vi "Dashboard Main.vi"() -> ()   [LabVIEW 2013]
uses:
  <vilib>/event_ctls.llb/eventvkey.ctl
  <vilib>/Rock Robotics/WPI/Dashboard/WPI_DashboardLogging Global.vi
  <vilib>/Utility/config.llb/Write Key (String).vi
  <vilib>/Utility/config.llb/Write Key (I32).vi
  <vilib>/Utility/config.llb/NI_LVConfig.lvlib
panel:
  out "Image Message":string="Timeout in Camera Communications"
  in  "Rec Mode":enum32{"Stop", "Record", "Playback"}(radio)
  in  "Dashboard Tab":T1(tab)
  out "Error":bool
  in  "Camera Settings":T2={"Frame Rate"=30, "Compression"=30, "Size"=1} {"Frame Rate" scale=1.0..30.0; "Size" items=["640x480", "320x240", "160x120"]}
  out "MotorSliders R":cluster{"MotorSlide1":dbl, "MotorSlide2":dbl} {"MotorSlide2" scale=-1.0..1.0 scale format="%#_2e"; "MotorSlide1" scale=-1.0..1.0 scale format="%#_2e"}
  out "MotorChart R":cluster{"Numeric":dbl, "Numeric":dbl}(graph)
  out "MotorSliders L":T3 {"MotorSlide4 2" scale=0.0..14.0 scale format="%#_2e"; "MotorSlide2" scale=-1.0..1.0 scale format="%#_2e"; "MotorSlide1" scale=-1.0..1.0 scale format="%#_2e"}
  out "MotorChart L":T4(graph)
  out "JS1 Z":dbl(slide) scale=-1.0..1.0 scale format="%#_2e"
  out "Joystick 1":cluster{"X":dbl, "Y":dbl}[](graph)
  out "JS Buttons 1":T5
  out "JS2 Z":dbl(slide) scale=-1.0..1.0 scale format="%#_2e"
  out "Joystick 2":cluster{"X":dbl, "Y":dbl}[](graph)
  out "JS Buttons 2":T5
  out "Mode":T6(ring)=enum."Auto Disabled"
  out "Camera IP":string
  in  "DB Camera Config":bool
  out "fps":dbl format="%#.1g"
  out "Mbps":dbl format="%#.1g"
  out "Mbps 2":bool
  in  "Test Slider":dbl(slide) scale=0.0..100.0 scale format="%#_3g"
  in  "On/Off":bool caption="Solenoid"
  in  "Test Name":u16(ring) items=["Select the test to run...", "Example Test", "-------------------------------", "List of tests is built in robot code.", "Replace with your own automated tests."]
  in  "Test Tree":string(tree)
  in  "Motor":cluster{"Value":dbl, "Enable":bool} {"Value" scale=-1.0..1.0 scale format="%#_3g"}
  out "Progress":T7 {"Test Progress" scale=0.0..100.0}
  in  "Rev/Fwd":cluster{"Forward":bool, "Reverse":bool}
  in  "Test Ring":u16(ring) items=["Auto", "Fixed indoor", "Fixed outdoor 1", "Fixed outdoor 2", "Fixed fluorescent 1", "Fixed fluorescent 2", "Hold current"]
  in  "Listbox":i32(listbox)
  out "Tree":string(tree)
  in  "Reset":bool
  out "Errors":T8(array[cluster])
  out "Camera Image":T9(plugin-control)
  in  "Enable":bool
  # "Left"
  # "Front"
  # "Right"
  # "Battery"
  # "Customize by placing controls and indicators here and name to\nmatch Dashboard Variables on robot."
  # "This tab is a great place for autonomous settings and validation.\nCustomize by placing controls and indicators here and name to\nmatch Dashboard Variables on robot."
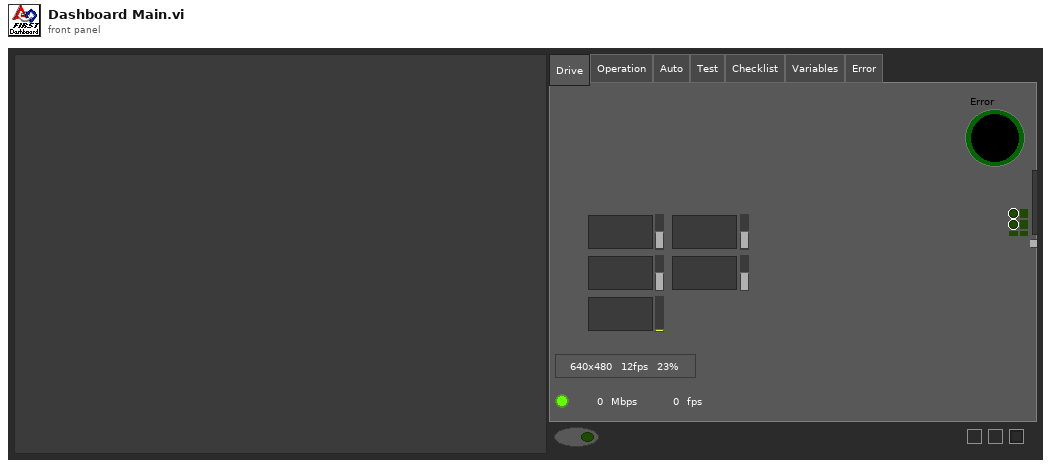
[diagram p1: front panel]
types:
  T1 = enum32{"Drive", "Operation", "Auto", "Test", "Checklist", "Variables", "Error"}
  T2 = cluster{"Frame Rate":i32, "Compression":i32, "Size":u16}
  T3 = cluster{"MotorSlide1":dbl, "MotorSlide2":dbl, "MotorSlide4 2":dbl}
  T4 = cluster{"Numeric":dbl, "Numeric":dbl, "Battery":sgl}
  T5 = cluster{bool, bool, bool, bool, bool, bool, bool, bool, bool, bool, bool, bool}
  T6 = enum8{"Tele-Op Disabled", "Tele-Op Enabled", "Auto Disabled", "Auto Enabled", "Test Disabled", "Test Enabled", ""}
  T7 = cluster{"Test Progress":u8, "Test Progress Text":string}
  T8 = cluster{"status":bool, "code":i32, "location":string, "source":string}[]
  T9 = typedef "IMAQ Image.ctl" = refnum<image>
  T10 = enum32{"Drive", "Operation", "Auto", "Test", "Checklist", "Variables"}
  T11 = typedef "Image Type" = u32
  T12 = cluster{"Digital Inputs":bool[], "Digital Outputs":bool[]}
  T13 = cluster{"Competition mode":bool, "Robot Link":bool, "Autonomous":bool, "Enabled":bool, "E-Stop":bool, "Simulated":bool, "TestMode":bool, "Docked Window":bool}
  T14 = cluster{"Boolean":bool, "Numeric":i32, "String":string, "String":string}[]
  T15 = typedef "NI_LVConfig.lvlib/Config Data RefNum.ctl" = refnum<k1>
  T16 = typedef "eventvkey.ctl" = enum16{"ASCII", "Enter", "Return", "Shift", "Ctrl", "Alt", "Cmd", "Opt", "Caps", "NumLock", "Clear", "Break", "Up", "Down", "Left", "Right", "Insert", "Delete", "Home", "End", "PageUp", "PageDown", "Escape", "Help", "Pause", "ScrollLock", "F1", "F2", "F3", "F4", "F5", "F6", "F7", "F8", "F9", "F10", "F11", "F12", "F13", "F14", "F15", "F16", "F17", "F18", "F19", "F20", "F21", "F22", "F23", "F24", "Play", "VolumeUp", "VolumeDown", "Mute", "Two Byte Char"}
  T17 = cluster{"Image Size":bool, "Image Type":bool, "Pixel Value":bool, "ROI Information":bool, "Zoom Factor":bool}
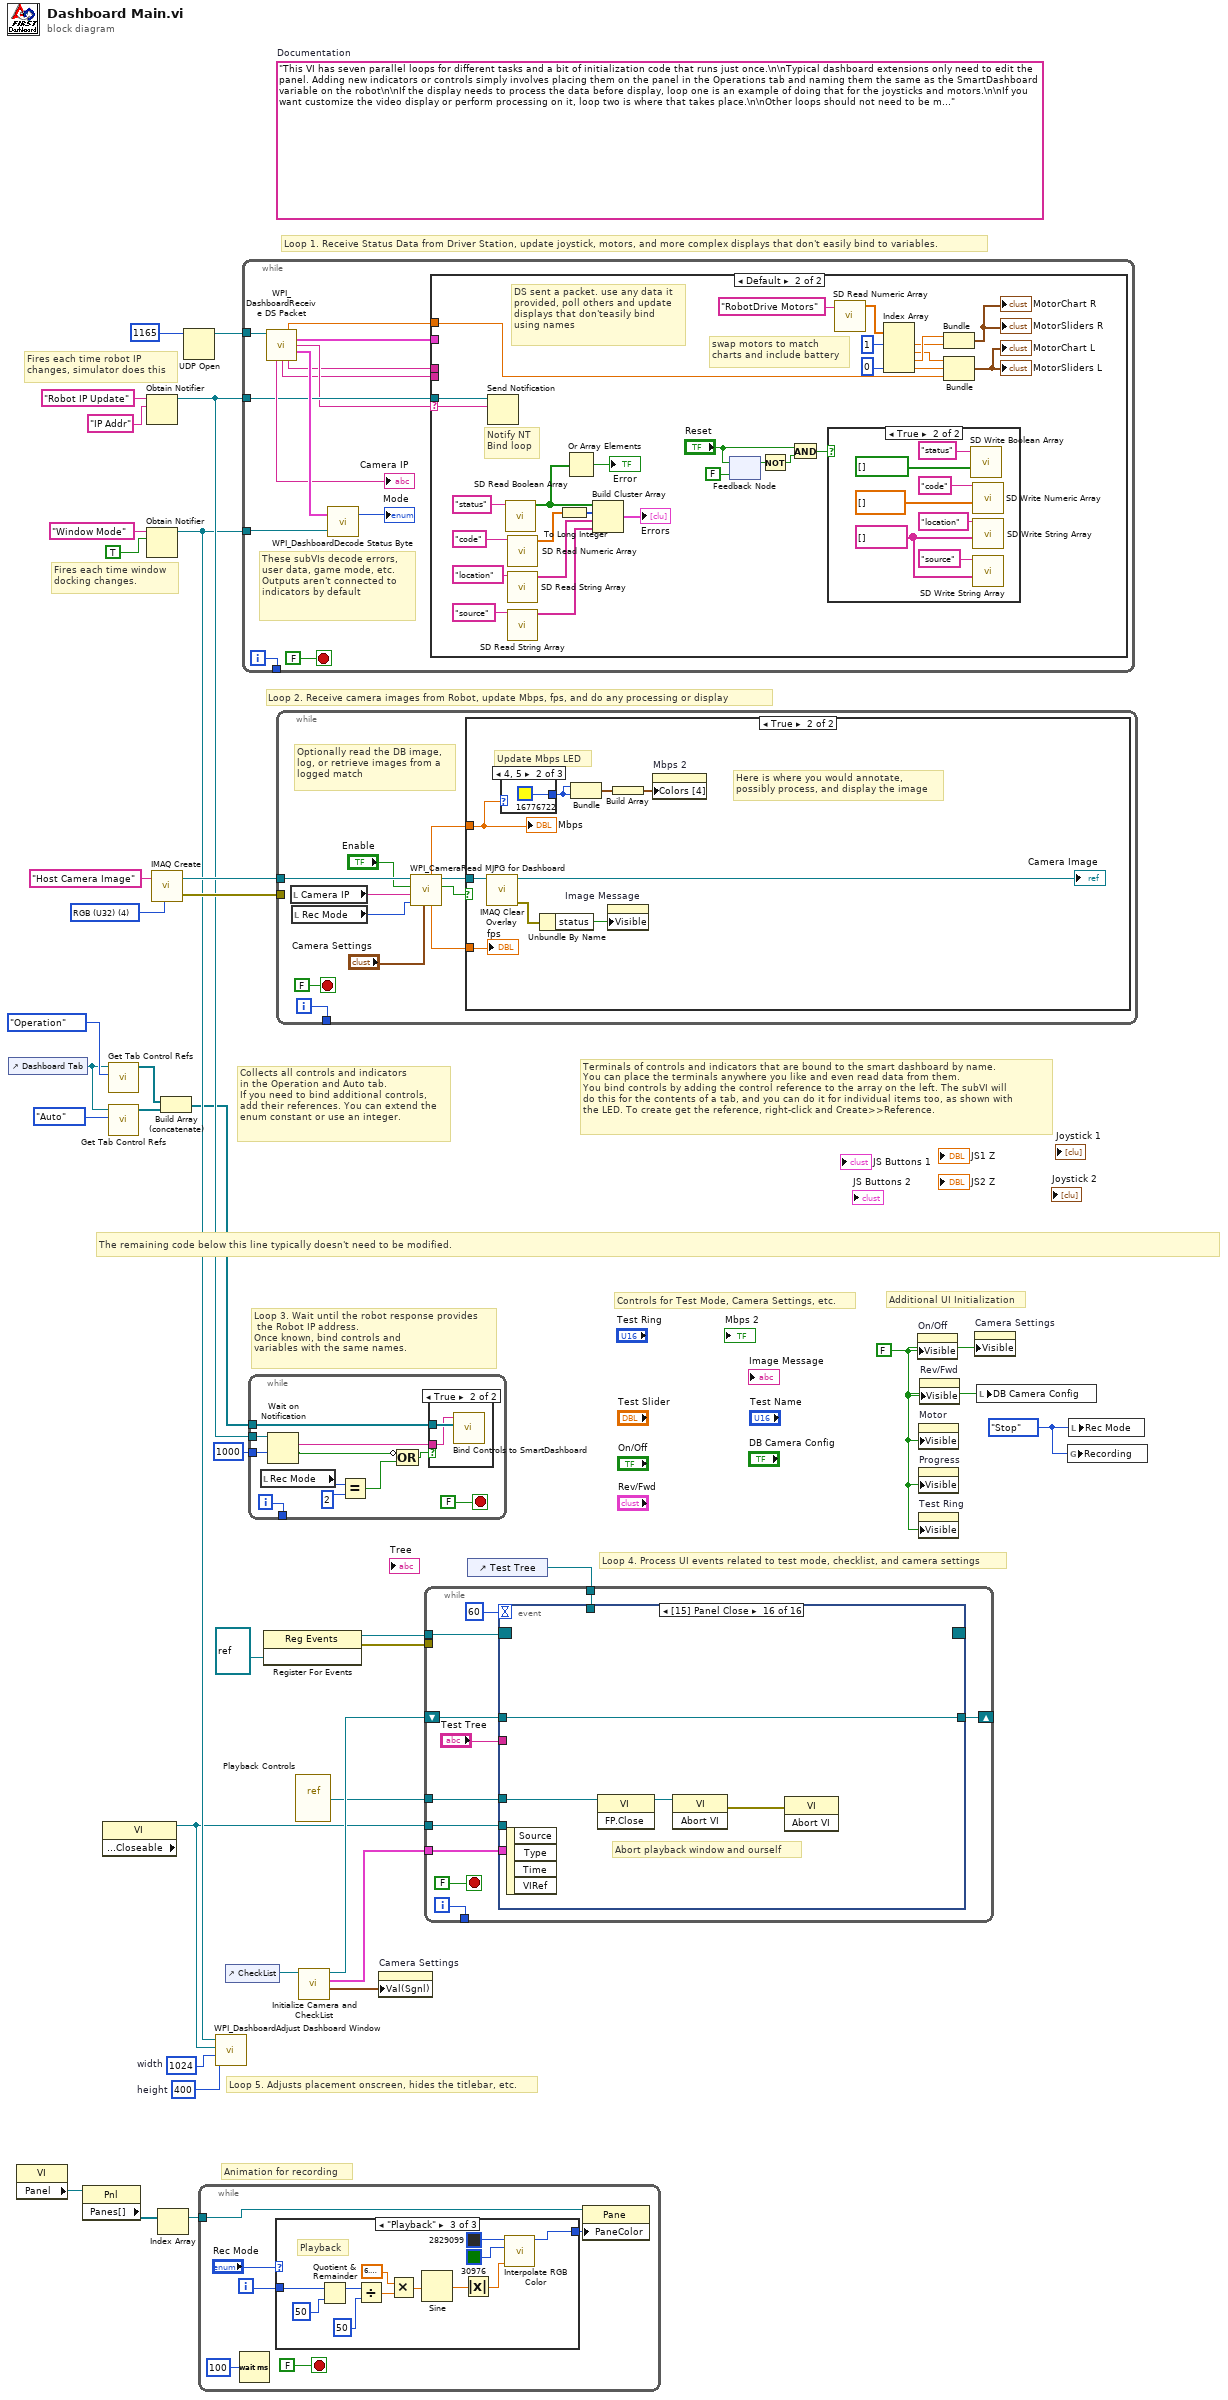
[diagram p0: block diagram]
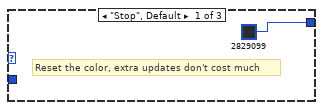
[diagram p2: hidden frame]
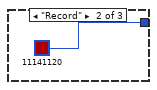
[diagram p3: hidden frame]
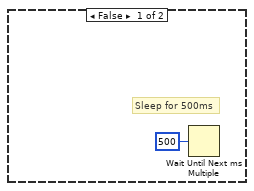
[diagram p5: hidden frame]
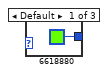
[diagram p6: hidden frame]
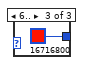
[diagram p7: hidden frame]
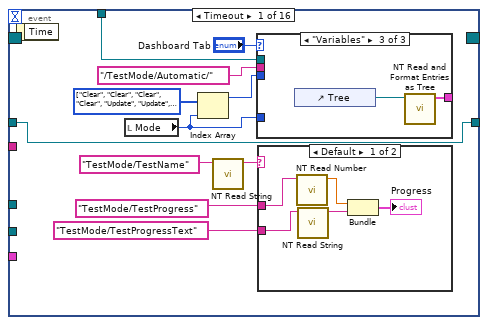
[diagram p8: hidden frame]
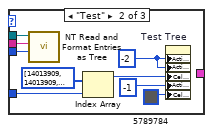
[diagram p10: hidden frame]
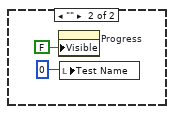
[diagram p11: hidden frame]
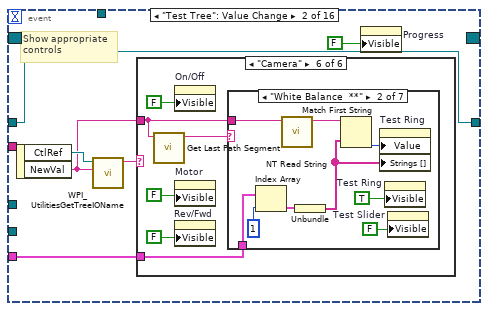
[diagram p12: hidden frame]
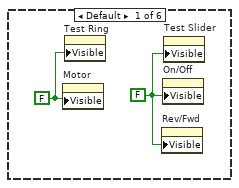
[diagram p13: hidden frame]
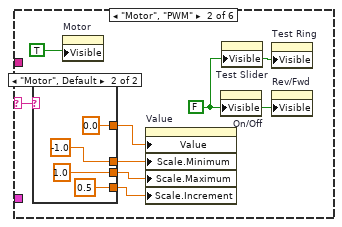
[diagram p14: hidden frame]
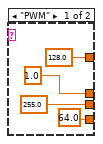
[diagram p15: hidden frame]
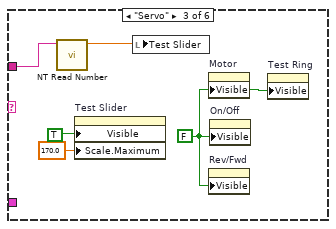
[diagram p16: hidden frame]
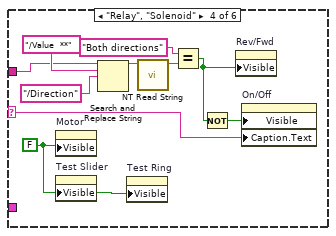
[diagram p17: hidden frame]
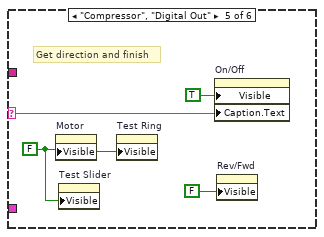
[diagram p18: hidden frame]
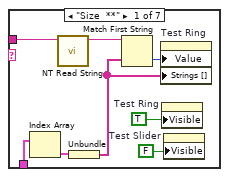
[diagram p19: hidden frame]
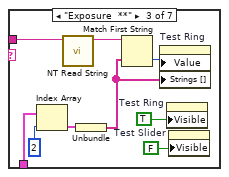
[diagram p20: hidden frame]
diagram:
  w7 = enum32{"Stop", "Record", "Playback"}."Stop" ("Rec Mode")
  w10 = 400  # height
  w11 = 1024  # width
  w24 = FALSE ("Visible")
  (unwired) "This VI has seven parallel loops for different tasks and a bit of initialization code that runs just once.\n\nTypical dashboard extensions only need to edit the panel. Adding new indicators or controls simply involves placing them on the panel in the Operations tab and naming them the same as the SmartDashboard variable on the robot\n\nIf the display needs to process the data before display, loop one is an example of doing that for the joysticks and motors.\n\nIf you want customize the video display or perform processing on it, loop two is where that takes place.\n\nOther loops should not need to be modified. They are pretty standard, and document the task they perform."  # Documentation
  w34 = T11 4 items=["Grayscale (U8)", "Grayscale (I16)", "Grayscale (SGL)", "Complex (CSG)", "RGB (U32)", "HSL (U32)", "RGB (U64)"] ("Image Type")
  # "Controls for Test Mode, Camera Settings, etc."
  # "Additional UI Initialization"
  # "Animation for recording"
  # "Fires each time robot IP\nchanges, simulator does this"
  # "Fires each time window\ndocking changes."
  # "Collects all controls and indicators\nin the Operation and Auto tab.\nIf you need to bind additional controls,\nadd their references. You can extend the\nenum constant or use an integer."
  # "The remaining code below this line typically doesn't need to be modified."
  # "Loop 4. Process UI events related to test mode, checklist, and camera settings"
  # "Terminals of controls and indicators that are bound to the smart dashboard by name.\nYou can place the terminals anywhere you like and even read data from them.\nYou bind controls by adding the control reference to the array on the left. The subVI will\ndo this for the contents of a tab, and you can do it for individual items too, as shown with\nthe LED. To create get the reference, right-click and Create>>Reference."
  # "Loop 3. Wait until the robot response provides\n the Robot IP address.\nOnce known, bind controls and\nvariables with the same names."
  # "Loop 5. Adjusts placement onscreen, hides the titlebar, etc."
  # "Loop 1. Receive Status Data from Driver Station, update joystick, motors, and more complex displays that don't easily bind to variables."
  # "Loop 2. Receive camera images from Robot, update Mbps, fps, and do any processing or display"
  n1 = control-ref of="Dashboard Tab"() -> (w5:refnum<vi>)
  n2 = property class="VI"() -> ("Panel"=w18:refnum<vi>)  [unwired: 2 in, 2 out]
  n3 = property class="Pnl"(reference=w18) -> ("Panes[]"=w19:refnum<vi>[])  [unwired: 1 in, 2 out]
  n4 = property class="VI" props=["Front Panel.Closeable"]() -> (reference out=w6:refnum<vi>)  [unwired: 2 in, 2 out]
  n5 = call <vilib>:"Get Tab Control Refs.vi"("Page Index"=T10."Operation" ("Dashboard Tab"), "TabControl in"=w5) -> ("ControlsOnPage"=w3:refnum<vi>[])  [unwired: 9 in]
  n6 = call <vilib>:"Get Tab Control Refs.vi"("Page Index"=T10."Auto" ("Dashboard Tab"), "TabControl in"=w5) -> ("ControlsOnPage"=w4:refnum<vi>[])  [unwired: 9 in]
  n7 = Obtain Notifier(name (unnamed)="Robot IP Update", notification data type="IP Addr" ("name (unnamed)")) -> (notifier out=w28:refnum<notifier>)  [unwired: 2 in, 2 out]
  n8 = Obtain Notifier(name (unnamed)="Window Mode", notification data type=TRUE) -> (notifier out=w9:refnum<notifier>)  [unwired: 2 in, 2 out]
  n9 = call "IMAQ Create"("Image Name"="Host Camera Image", "Image Type"=w34) -> ("New Image"=w32:T9, "error out"=w31:errorcluster)  [unwired: 2 in, 1 out]
  n10 = Index Array(array=w19) -> (element=w17:refnum<vi>)  [unwired: 1 in]
  n11 = Build Array (concatenate)(w3, w4) -> (w2:refnum<vi>[])
  n12 = UDP Open(11:u16 1165 ("port")) -> (port=w35:refnum<k16>)  [unwired: 2 in, 4 out]
  n13 = while {
    tunnel: w17 -> [w38]
    i -> [w41]
    stop <- FALSE stop-if-true
    n14 = Wait (ms)(milliseconds to wait=u32 100) -> ()  [unwired: 1 out]
    n15 = case shown="\"Playback\"" "Rec Mode" {
      tunnel: w41 -> [_ _ w56]
      tunnel: [u32 2829099 ("Base Color") u32 11141120 ("Target Color") w45] -> w37
      frame "Stop", Default {
        # "Reset the color, extra updates don't cost much"
      }
      frame "Record" {
      }
      frame "Playback" {
        # "Playback"
        n16 = Quotient & Remainder(x=w56, y=u32 50 ("milliseconds to wait")) -> (x-y*floor(x/y)=w52:u32)  [unwired: 1 out]
        n17 = Divide(x=w52, y=u32 50 ("milliseconds to wait")) -> (x/y=w49:dbl)
        n18 = Multiply(x=6.283185307179586, y=w49) -> (x*y=w54:dbl)
        n19 = Sine(x=w54) -> (sin(x)=w53:dbl)
        n20 = Absolute Value(x=w53) -> (abs(x)=w46:dbl)
        n21 = call "Interpolate RGB Color.vi"("Proportion"=w46, "Target Color"=u32 30976, "Base Color"=u32 2829099) -> ("Result Color"=w45:u32)  [unwired: 8 in]
      }
    }
    n22 = property class="Pane"(reference=w38, "PaneColor"=w37) -> ()  [unwired: 1 in, 2 out]
  }
  n23 = call <vilib>:"WPI_DashboardAdjust Dashboard Window.vi"("height"=w10, "width"=w11, "reference in"=w6, "Notifier in"=w9) -> ()  [unwired: 8 in]
  n24 = control-ref of="CheckList"() -> (w8:refnum<vi>)
  n25 = while {
    tunnel: w35 -> [w67]
    tunnel: w28 -> [w62]
    tunnel: w9 -> [w66]
    tunnel: [w63] -> _
    i -> [w63]
    stop <- FALSE stop-if-true
    # "These subVIs decode errors, user data, game mode, etc.\nOutputs aren't connected to indicators by default"
    n26 = call <vilib>:"WPI_DashboardReceive DS Packet.vi"("Recv Socket"=w67) -> ("Battery"=w57:sgl, "Driver Station"=w58:T12, "Robot IP Address"=w61:string, "Status"=w68:T13, "Camera IP Address"=→"Camera IP":string, "Low Priority User Data"=w60:string, "High Priority User Data"=w59:string)  [unwired: 1 in, 7 out]
    n27 = call <vilib>:"WPI_DashboardDecode Status Byte.vi"("Window Mode Notifier"=w66, "Status"=w68) -> ("Mode"=→"Mode":T6)  [unwired: 1 out]
    n28 = case shown="Default" w61 {
      selector: w61 -> [_ w96]
      tunnel: w62 -> [_ w97]
      tunnel: w60 -> [_ _]
      tunnel: w59 -> [_ _]
      tunnel: w58 -> [_ _]
      tunnel: w57 -> [_ w95]
      frame "0.0.0.0" {
        # "DS not sending packets, or no robot exists yet.\nDon't poll the variables"
      }
      frame Default {
        # "Notify NT\nBind loop"
        # "DS sent a packet. use any data it\nprovided, poll others and update\ndisplays that don'teasily bind\nusing names"
        # "swap motors to match\ncharts and include battery"
        n29 = Send Notification(notification=w96, notifier=w97) -> ()  [unwired: 1 in, 2 out]
        n30 = call <vilib>:"SD Read Boolean Array.vi"("Name"="status") -> ("Boolean Array"=w74:bool[])  [unwired: 8 in, 2 out]
        n31 = call <vilib>:"SD Read Numeric Array.vi"("Name"="code") -> ("Numeric Array"=w73:dbl[])  [unwired: 8 in, 2 out]
        n32 = call <vilib>:"SD Read String Array.vi"("Name"="location") -> ("String Array"=w72:string[])  [unwired: 9 in, 1 out]
        n33 = call <vilib>:"SD Read String Array.vi"("Name"="source") -> ("String Array"=w71:string[])  [unwired: 9 in, 1 out]
        n34 = To Long Integer(number=w73) -> (32bit integer=w85:i32[])
        n35 = Or Array Elements(Boolean array=w74) -> (logical OR=→"Error":bool)
        n36 = Build Cluster Array(w74, w85, w72, w71) -> (→"Errors":T14)
        n37 = feedback-in #1("Reset") -> ()
        n38 = feedback #1(FALSE ("Reset")) -> (w77:bool)
        n39 = Not(x=w77) -> (.not. x?=w76:bool)
        n40 = And(x="Reset", y=w76) -> (x .and. y?=w70:bool)
        n41 = case shown="True" w70 {
          frame False {
          }
          frame True {
            w99 = string[] [] ("String Array")
            n42 = call <vilib>:"SD Write Boolean Array.vi"("Boolean Array"=bool[] [], "Name"="status") -> ()  [unwired: 8 in, 2 out]
            n43 = call <vilib>:"SD Write Numeric Array.vi"("Numeric Array"=dbl[] [], "Name"="code") -> ()  [unwired: 8 in, 2 out]
            n44 = call <vilib>:"SD Write String Array.vi"("String Array"=w99, "Name"="location") -> ()  [unwired: 8 in, 2 out]
            n45 = call <vilib>:"SD Write String Array.vi"("String Array"=w99, "Name"="source") -> ()  [unwired: 8 in, 2 out]
          }
        }
        n46 = call <vilib>:"SD Read Numeric Array.vi"("Name"="RobotDrive Motors") -> ("Numeric Array"=w94:dbl[])  [unwired: 8 in, 2 out]
        n47 = Index Array(array=w94, index #1=1, index #4=0) -> (element #1=w90:dbl, element #2=w89:dbl, element #3=w91:dbl, element #4=w86:dbl)  [unwired: 2 in]
        n48 = Bundle("Numeric"=w91, "Numeric"=w90) -> (→"MotorChart R" →"MotorSliders R":cluster{"Numeric":dbl, "Numeric":dbl})  [unwired: 1 in]
        n49 = Bundle("Numeric"=w89, "Numeric"=w86, "Battery"=w95) -> (→"MotorChart L" →"MotorSliders L":T4)  [unwired: 1 in]
      }
    }
  }
  n50 = while {
    tunnel: w2 -> [w116]
    tunnel: w28 -> [w114]
    tunnel: [w112] -> _
    tunnel: u32 1000 ("milliseconds to wait") -> [w111]
    i -> [w112]
    stop <- FALSE stop-if-true
    n51 = local read "Rec Mode"() -> (w107:enum32{"Stop", "Record", "Playback"})
    n52 = Wait on Notification(notifier=w114, timeout in ms (-1)=w111) -> (notification=w113:string, timed out?=w109:bool)  [unwired: 2 in, 2 out]
    n53 = Equal?(x=w107, y=u16 2 ("Rec Mode")) -> (x = y?=w108:bool)
    n54 = Compound Arithmetic op=OR(invert w109, w108) -> (w110:bool)
    n55 = case shown="True" w110 {
      tunnel: w116 -> [_ w118]
      tunnel: w113 -> [_ w117]
      frame False {
      }
      frame True {
        n56 = call <vilib>:"Bind Controls to SmartDashboard.vi"("Bound Control Refs"=w118, "Server IP Address"=w117) -> ()  [unwired: 10 in]
      }
    }
  }
  n57 = register-events(refnum<vi> refnum) -> (reference out=w15:refnum<event-registration>, error out=w14:errorcluster)  [unwired: 2 in]
  n58 = while {
    tunnel: w32 -> [w127]
    tunnel: w31 -> [_]
    tunnel: [w128] -> _
    i -> [w128]
    stop <- FALSE stop-if-true
    # "Optionally read the DB image,\nlog, or retrieve images from a\nlogged match"
    n59 = local read "Camera IP"() -> (w120:string)
    n60 = local read "Rec Mode"() -> (w119:enum32{"Stop", "Record", "Playback"})
    n61 = call <vilib>:"WPI_CameraRead MJPG for Dashboard.vi"("Camera Settings"="Camera Settings", "Rec Mode"=w119, "Camera IP"=w120, "Enable"="Enable", "Refnum in"=w127) -> ("Active"=w124:bool, "Refnum out"=w126:T9, "FPS"=w123:dbl, "Bandwidth (Mbps)"=w122:dbl)  [unwired: 3 in]
    n62 = case shown="True" w124 {
      tunnel: w126 -> [_ w134]
      tunnel: w122 -> [_ w133]
      tunnel: w123 -> [_ w131]
      frame False {
        # "Sleep for 500ms"
        n63 = Wait Until Next ms Multiple(millisecond multiple=u32 500) -> ()  [unwired: 1 out]
      }
      frame True {
        # "Here is where you would annotate,\npossibly process, and display the image"
        # "Update Mbps LED"
        n64 = call "IMAQ Clear Overlay"("Image"=w134) -> ("error out"=w138:errorcluster, "Image Out"=→"Camera Image":T9)  [unwired: 2 in, 7 out]
        n65 = case shown="4, 5" w133 {
          tunnel: [u32 6618880 ("Color Box") u32 16776722 ("Color Box") u32 16716800 ("Color Box")] -> w135
          frame Default {
          }
          frame 4, 5 {
          }
          frame 6.. {
          }
        }
        n66 = Unbundle By Name(w138) -> ("status"=w139:bool)
        n67 = Bundle("Color Box"=w135, "Color Box"=w135) -> (w137:cluster{"Color Box":u32, "Color Box":u32})  [unwired: 1 out]
        n68 = property on="Image Message" class="Str"("Visible"=w139) -> ()  [unwired: 2 in, 2 out]
        n69 = Build Array(w137) -> (w136:cluster{"Color Box":u32, "Color Box":u32}[])
        n70 = property on="Mbps 2" class="Bool (strict)"("Colors [4]"=w136) -> ()  [unwired: 2 in, 2 out]
        "Mbps" <- w133
        "fps" <- w131
      }
    }
  }
  n71 = vi-ref "Playback Controls.vi"() -> (w16:refnum<vi>)
  n72 = call "Initialize Camera and CheckList.vi"("ListBox in"=w8) -> ("Cluster"=w22:cluster{"value":i32, "value":i32, "index":i32}, "Array"=w23:cluster{string[]}[], "File Refnum"=w21:T15)  [unwired: 8 in]
  n73 = property on="Camera Settings" class="Clust (strict)"("Val(Sgnl)"=w22) -> ()  [unwired: 2 in, 2 out]
  n74 = control-ref of="Test Tree"() -> (w20:refnum<vi>)
  n75 = while {
    tunnel: w23 -> [w150]
    shift-right: [w149] -> _
    shift-left: w21 -> [w148]
    tunnel: [w147] -> _
    tunnel: w20 -> [w146]
    tunnel: w16 -> [w145]
    tunnel: w15 -> [w144]
    tunnel: w14 -> [_]
    tunnel: w6 -> [w143]
    i -> [w147]
    stop <- FALSE stop-if-true
    n76 = event shown="[15] Panel Close" {
      selector: w144 -> [_ _ _ _ _ _ _ _ _ _ _ _ _ _ _ _]
      dyn-events: [_ _ _ _ _ _ _ _ _ _ _ _ _ w388 _ _] -> _
      timeout: u32 60 ("milliseconds to wait") -> [_ _ _ _ _ _ _ _ _ _ _ _ _ _ _ _]
      tunnel: w146 -> [w160 _ _ _ _ _ _ _ _ _ _ _ _ _ _ _]
      tunnel: "Test Tree" -> [_ _ _ _ _ _ _ _ w357 w365 w367 w371 w379 _ _ _]
      tunnel: w150 -> [_ w184 _ _ _ _ w321 w351 _ _ _ _ _ _ _ _]
      tunnel: [w154 w183 w282 w287 w295 w307 w320 w344 w356 w363 w366 w370 w378 w390 w404 w405] -> w149
      tunnel: w148 -> [w154 w183 w282 w287 w295 w307 w319 w344 w356 w363 w366 w370 w378 w390 w404 w405]
      tunnel: w145 -> [_ _ _ _ _ _ _ _ _ _ _ _ _ w391 _ w408]
      tunnel: w143 -> [_ _ _ _ _ _ _ _ _ _ _ _ _ w386 _ _]
      event Timeout {
        w159 = enum16{"Update", "Clear"}[] [enum."Clear", enum."Clear", enum."Clear", enum."Clear", enum."Update", enum."Update", enum."Clear"] items=["Update", "Clear"]
        n77 = event-data() -> ()  [unwired: 1 in, 1 out]
        n78 = local read "Mode"() -> (w157:T6)
        n79 = Index Array(array=w159, index=w157) -> (element=w158:enum16{"Update", "Clear"})
        n80 = call <vilib>:"NT Read String.vi"("Name"="TestMode/TestName") -> ("String"=w163:string)  [unwired: 9 in, 1 out]
        n81 = case shown="\"Variables\"" "Dashboard Tab" {
          tunnel: w160 -> [_ w173 _]
          tunnel: "/TestMode/Automatic/" ("Name Pattern") -> [_ w172 _]
          tunnel: w158 -> [_ w171 _]
          tunnel: w157 -> [_ w169 _]
          tunnel: [_ _ w175] -> _
          frame "Operation", Default {
          }
          frame "Test" {
            w168 = -2 ("Active Item:Row Number")
            n82 = call <vilib>:"NT Read and Format Entries as Tree.vi"("Operation"=w171, "Name Pattern"=w172, "Tree Refnum"=w173) -> ()  [unwired: 7 in, 2 out]
            n83 = Index Array(array=u32[] [14013909, 14013909, 14013909, 14013909, 14013909, 16777215, 14013909], index=w169) -> (element=w167:u32)
            n84 = property on="Test Tree" class="Tree (strict)"("Active Item Row Number"=w168, "ActiveColNum"=w168, "CellBG"=w167, "Active Item Row Number"=-1 ("Active Item:Row Number"), "CellBG"=u32 5789784 ("Color Box")) -> ()  [unwired: 2 in, 2 out]
          }
          frame "Variables" {
            n85 = control-ref of="Tree"() -> (w174:refnum<vi>)
            n86 = call <vilib>:"NT Read and Format Entries as Tree.vi"("Tree Refnum"=w174) -> ("Formatted Strings"=w175:cluster{"Name":string, "Value":string}[])  [unwired: 9 in, 1 out]
          }
        }
        n87 = case shown="Default" w163 {
          tunnel: "TestMode/TestProgress" ("Name") -> [w177 _]
          tunnel: "TestMode/TestProgressText" ("Name") -> [w176 _]
          frame Default {
            n88 = call <vilib>:"NT Read Number.vi"("Name"=w177) -> ("Numeric"=w178:dbl)  [unwired: 9 in, 1 out]
            n89 = call <vilib>:"NT Read String.vi"("Name"=w176) -> ("String"=w179:string)  [unwired: 9 in, 1 out]
            n90 = Bundle("Numeric"=w178, "String"=w179) -> (→"Progress":cluster{"Numeric":dbl, "String":string})  [unwired: 1 in]
          }
          frame "" {
            n91 = property on="Progress" class="Clust (strict)"("Visible"=FALSE) -> ()  [unwired: 2 in, 2 out]
            n92 = local write "Test Name"(u16 0) -> ()
          }
        }
      }
      event "Test Tree": Value Change {
        # "Show appropriate\ncontrols"
        n93 = event-data() -> ("CtlRef"=w187:refnum<vi>, "NewVal"=w185:string)  [unwired: 1 in]
        n94 = call <vilib>:"WPI_UtilitiesGetTreeIOName.vi"("NewVal"=w185, "TreeControl in"=w187) -> ("I/O Name"=w188:string)  [unwired: 9 in]
        n95 = case shown="\"Camera\"" w188 {
          selector: w188 -> [_ w195 _ w213 w222 _]
          tunnel: w185 -> [_ _ w210 w212 _ w229]
          tunnel: w184 -> [_ _ _ _ _ w228]
          frame Default {
            w190 = FALSE ("Visible")
            w189 = FALSE ("Visible")
            n96 = property on="Motor" class="Clust (strict)"("Visible"=w189) -> ()  [unwired: 2 in, 2 out]
            n97 = property on="Test Ring" class="Ring (strict)"("Visible"=w189) -> ()  [unwired: 2 in, 2 out]
            n98 = property on="Rev/Fwd" class="Clust (strict)"("Visible"=w190) -> ()  [unwired: 2 in, 2 out]
            n99 = property on="On/Off" class="Bool (strict)"("Visible"=w190) -> ()  [unwired: 2 in, 2 out]
            n100 = property on="Test Slider" class="Slide (strict)"("Visible"=w190) -> ()  [unwired: 2 in, 2 out]
          }
          frame "Motor", "PWM" {
            w196 = FALSE ("Visible")
            n101 = case shown="\"Motor\", Default" w195 {
              tunnel: [1.0 ("Value") -1.0 ("Value")] -> w194
              tunnel: [255.0 ("Value") 1.0 ("Value")] -> w193
              tunnel: [128.0 ("Value") 0.0 ("Value")] -> w192
              tunnel: [64.0 ("Value") 0.5 ("Value")] -> w191
              frame "PWM" {
              }
              frame "Motor", Default {
              }
            }
            n102 = property on="Motor" class="Clust (strict)"("Visible"=TRUE) -> ()  [unwired: 2 in, 2 out]
            n103 = property on="Value" class="Slide (strict)"("Value"=w192, "Scale.Minimum"=w194, "Scale.Maximum"=w193, "Scale.Increment"=w191) -> ()  [unwired: 2 in, 2 out]
            n104 = property on="On/Off" class="Bool (strict)"("Visible"=w196) -> ()  [unwired: 2 in, 2 out]
            n105 = property on="Test Slider" class="Slide (strict)"("Visible"=w196) -> ()  [unwired: 2 in, 2 out]
            n106 = property on="Test Ring" class="Ring (strict)"("Visible"=w196) -> ()  [unwired: 2 in, 2 out]
            n107 = property on="Rev/Fwd" class="Clust (strict)"("Visible"=w196) -> ()  [unwired: 2 in, 2 out]
          }
          frame "Servo" {
            w208 = FALSE ("Visible")
            n108 = call <vilib>:"NT Read Number.vi"("Name"=w210) -> ("Numeric"=w209:dbl)  [unwired: 9 in, 1 out]
            n109 = property on="Test Slider" class="Slide (strict)"("Visible"=TRUE, "Scale.Maximum"=170.0 ("Scale.Range:Maximum")) -> ()  [unwired: 2 in, 2 out]
            n110 = local write "Test Slider"(w209) -> ()
            n111 = property on="Motor" class="Clust (strict)"("Visible"=w208) -> ()  [unwired: 2 in, 2 out]
            n112 = property on="Rev/Fwd" class="Clust (strict)"("Visible"=w208) -> ()  [unwired: 2 in, 2 out]
            n113 = property on="On/Off" class="Bool (strict)"("Visible"=w208) -> ()  [unwired: 2 in, 2 out]
            n114 = property on="Test Ring" class="Ring (strict)"("Visible"=w208) -> ()  [unwired: 2 in, 2 out]
          }
          frame "Relay", "Solenoid" {
            w211 = FALSE ("Visible")
            n115 = property on="Motor" class="Clust (strict)"("Visible"=w211) -> ()  [unwired: 2 in, 2 out]
            n116 = property on="Test Slider" class="Slide (strict)"("Visible"=w211) -> ()  [unwired: 2 in, 2 out]
            n117 = Search and Replace String(input string=w212, search string="/Value  **", replace string="/Direction") -> (result string=w218:string)  [unwired: 5 in, 3 out]
            n118 = property on="Test Ring" class="Ring (strict)"("Visible"=w211) -> ()  [unwired: 2 in, 2 out]
            n119 = call <vilib>:"NT Read String.vi"("Name"=w218) -> ("String"=w216:string)  [unwired: 9 in, 1 out]
            n120 = Equal?(x="Both directions", y=w216) -> (x = y?=w214:bool)
            n121 = Not(x=w214) -> (.not. x?=w215:bool)
            n122 = property on="Rev/Fwd" class="Clust (strict)"("Visible"=w214) -> ()  [unwired: 2 in, 2 out]
            n123 = property on="On/Off" class="Bool (strict)"("Visible"=w215, "Caption.Text"=w213) -> ()  [unwired: 2 in, 2 out]
          }
          frame "Compressor", "Digital Out" {
            w221 = FALSE ("Visible")
            # "Get direction and finish"
            n124 = property on="Motor" class="Clust (strict)"("Visible"=w221) -> ()  [unwired: 2 in, 2 out]
            n125 = property on="Test Slider" class="Slide (strict)"("Visible"=w221) -> ()  [unwired: 2 in, 2 out]
            n126 = property on="Test Ring" class="Ring (strict)"("Visible"=w221) -> ()  [unwired: 2 in, 2 out]
            n127 = property on="On/Off" class="Bool (strict)"("Visible"=TRUE, "Caption.Text"=w222) -> ()  [unwired: 2 in, 2 out]
            n128 = property on="Rev/Fwd" class="Clust (strict)"("Visible"=FALSE) -> ()  [unwired: 2 in, 2 out]
          }
          frame "Camera" {
            n129 = call <vilib>:"Get Last Path Segment.vi"("String in"=w229) -> ("String out"=w230:string)  [unwired: 10 in]
            n130 = property on="On/Off" class="Bool (strict)"("Visible"=FALSE) -> ()  [unwired: 2 in, 2 out]
            n131 = property on="Motor" class="Clust (strict)"("Visible"=FALSE) -> ()  [unwired: 2 in, 2 out]
            n132 = property on="Rev/Fwd" class="Clust (strict)"("Visible"=FALSE) -> ()  [unwired: 2 in, 2 out]
            n133 = case shown="\"White Balance  **\"" w230 {
              tunnel: w229 -> [w236 w245 w254 w263 w272 _ w278]
              tunnel: w228 -> [w234 w242 w251 w260 w269 _ _]
              frame "Size  **" {
                n134 = Index Array(array=w234) -> (element=w233:cluster{string[]})  [unwired: 1 in]
                n135 = call <vilib>:"NT Read String.vi"("Name"=w236) -> ("String"=w235:string)  [unwired: 9 in, 1 out]
                n136 = Unbundle(w233) -> (w231:string[])
                n137 = Match First String(2:w231, 3:w235) -> (0:w232:i32)  [unwired: 1 out]
                n138 = property on="Test Ring" class="Ring (strict)"("Value"=w232, "Strings []"=w231) -> ()  [unwired: 2 in, 2 out]
                n139 = property on="Test Ring" class="Ring (strict)"("Visible"=TRUE) -> ()  [unwired: 2 in, 2 out]
                n140 = property on="Test Slider" class="Slide (strict)"("Visible"=FALSE) -> ()  [unwired: 2 in, 2 out]
              }
              frame "White Balance  **" {
                n141 = Index Array(array=w242, index=1) -> (element=w243:cluster{string[]})
                n142 = call <vilib>:"NT Read String.vi"("Name"=w245) -> ("String"=w244:string)  [unwired: 9 in, 1 out]
                n143 = Unbundle(w243) -> (w240:string[])
                n144 = Match First String(2:w240, 3:w244) -> (0:w239:i32)  [unwired: 1 out]
                n145 = property on="Test Ring" class="Ring (strict)"("Value"=w239, "Strings []"=w240) -> ()  [unwired: 2 in, 2 out]
                n146 = property on="Test Ring" class="Ring (strict)"("Visible"=TRUE) -> ()  [unwired: 2 in, 2 out]
                n147 = property on="Test Slider" class="Slide (strict)"("Visible"=FALSE) -> ()  [unwired: 2 in, 2 out]
              }
              frame "Exposure  **" {
                n148 = Index Array(array=w251, index=2) -> (element=w252:cluster{string[]})
                n149 = call <vilib>:"NT Read String.vi"("Name"=w254) -> ("String"=w253:string)  [unwired: 9 in, 1 out]
                n150 = Unbundle(w252) -> (w248:string[])
                n151 = Match First String(2:w248, 3:w253) -> (0:w249:i32)  [unwired: 1 out]
                n152 = property on="Test Ring" class="Ring (strict)"("Value"=w249, "Strings []"=w248) -> ()  [unwired: 2 in, 2 out]
                n153 = property on="Test Ring" class="Ring (strict)"("Visible"=TRUE) -> ()  [unwired: 2 in, 2 out]
                n154 = property on="Test Slider" class="Slide (strict)"("Visible"=FALSE) -> ()  [unwired: 2 in, 2 out]
              }
              frame "Exposure Priority  **" {
                n155 = Index Array(array=w260, index=3) -> (element=w261:cluster{string[]})
                n156 = call <vilib>:"NT Read String.vi"("Name"=w263) -> ("String"=w262:string)  [unwired: 9 in, 1 out]
                n157 = Unbundle(w261) -> (w257:string[])
                n158 = Match First String(2:w257, 3:w262) -> (0:w258:i32)  [unwired: 1 out]
                n159 = property on="Test Ring" class="Ring (strict)"("Value"=w258, "Strings []"=w257) -> ()  [unwired: 2 in, 2 out]
                n160 = property on="Test Ring" class="Ring (strict)"("Visible"=TRUE) -> ()  [unwired: 2 in, 2 out]
                n161 = property on="Test Slider" class="Slide (strict)"("Visible"=FALSE) -> ()  [unwired: 2 in, 2 out]
              }
              frame "Color Enable  **" {
                n162 = Index Array(array=w269, index=4) -> (element=w270:cluster{string[]})
                n163 = call <vilib>:"NT Read String.vi"("Name"=w272) -> ("String"=w271:string)  [unwired: 9 in, 1 out]
                n164 = Unbundle(w270) -> (w266:string[])
                n165 = Match First String(2:w266, 3:w271) -> (0:w267:i32)  [unwired: 1 out]
                n166 = property on="Test Ring" class="Ring (strict)"("Value"=w267, "Strings []"=w266) -> ()  [unwired: 2 in, 2 out]
                n167 = property on="Test Ring" class="Ring (strict)"("Visible"=TRUE) -> ()  [unwired: 2 in, 2 out]
                n168 = property on="Test Slider" class="Slide (strict)"("Visible"=FALSE) -> ()  [unwired: 2 in, 2 out]
              }
              frame Default {
                n169 = property on="Test Ring" class="Ring (strict)"("Visible"=FALSE) -> ()  [unwired: 2 in, 2 out]
                n170 = property on="Test Slider" class="Slide (strict)"("Visible"=FALSE) -> ()  [unwired: 2 in, 2 out]
              }
              frame "Brightness  **", "Color Level  **", "Compression  **", "FPS  **", "Sharpness  **" {
                n171 = call <vilib>:"NT Read Number.vi"("Name"=w278) -> ("Numeric"=w277:dbl)  [unwired: 9 in, 1 out]
                n172 = local write "Test Slider"(w277) -> ()
                n173 = property on="Test Slider" class="Slide (strict)"("Visible"=TRUE, "Scale.Maximum"=100.0 ("Scale.Range:Maximum")) -> ()  [unwired: 2 in, 2 out]
                n174 = property on="Test Ring" class="Ring (strict)"("Visible"=FALSE) -> ()  [unwired: 2 in, 2 out]
              }
            }
          }
        }
        n175 = property on="Progress" class="Clust (strict)"("Visible"=FALSE) -> ()  [unwired: 2 in, 2 out]
      }
      event "Test Name": Mouse Enter {
        # "Populate the ring with the list of tests"
        n176 = event-data() -> ()  [unwired: 1 in, 1 out]
        n177 = call <vilib>:"NT Read String Array.vi"("Name"="TestMode/TestList") -> ("String Array"=w286:string[])  [unwired: 9 in, 1 out]
        n178 = Build Array (concatenate)("Select the test to run...", w286) -> (w285:string[])
        n179 = property on="Test Name" class="Ring (strict)"("Strings []"=w285) -> ()  [unwired: 2 in, 2 out]
      }
      event "Test Name": Value Change {
        w288 = FALSE ("Visible")
        # "Tell the robot the test name to run"
        n180 = event-data() -> ("NewVal"=w292:u16)  [unwired: 1 in]
        n181 = property on="Test Name" class="Ring (strict)"() -> ("Strings []"=w293:string[])  [unwired: 2 in, 2 out]
        n182 = local write "Progress"(T7 {"Test Progress"=0, "Test Progress Text"=""} ("Progress")) -> ()
        n183 = Index Array(array=w293, index=w292) -> (element=w291:string)
        n184 = call <vilib>:"NT Write String.vi"("String"=w291, "Name"="TestMode/TestName") -> ()  [unwired: 9 in, 1 out]
        n185 = property on="Progress" class="Clust (strict)"("Visible"=TRUE) -> ()  [unwired: 2 in, 2 out]
        n186 = property on="Motor" class="Clust (strict)"("Visible"=w288) -> ()  [unwired: 2 in, 2 out]
        n187 = property on="Test Slider" class="Slide (strict)"("Visible"=w288) -> ()  [unwired: 2 in, 2 out]
        n188 = property on="On/Off" class="Bool (strict)"("Visible"=w288) -> ()  [unwired: 2 in, 2 out]
        n189 = property on="Rev/Fwd" class="Clust (strict)"("Visible"=w288) -> ()  [unwired: 2 in, 2 out]
        n190 = property on="Test Ring" class="Ring (strict)"("Visible"=w288) -> ()  [unwired: 2 in, 2 out]
      }
      event "Listbox": Double Click {
        n191 = event-data() -> ("PlatMods.Shift"=w296:bool, "Row"=w298:i32)  [unwired: 1 in]
        n192 = case shown="True" w296 {
          tunnel: w298 -> [w302 _]
          tunnel: 1 -> [w301 _]
          frame False {
            n193 = property on="Listbox" class="LstBox (strict)"() -> ("Item Symbols"=w300:i32[])  [unwired: 2 in, 2 out]
            n194 = Replace Array Subset(array=w300, new element=w301, index=w302) -> (w299:i32[])
            n195 = property on="Listbox" class="LstBox (strict)"("Item Symbols"=w299) -> ()  [unwired: 2 in, 2 out]
          }
          frame True {
            w303 = 0 ("Top Row")
            n196 = property on="Listbox" class="LstBox (strict)"() -> ("Number of Rows"=w305:u32)  [unwired: 2 in, 2 out]
            n197 = Initialize Array(0, w305) -> (w304:i32[])
            n198 = property on="Listbox" class="LstBox (strict)"("Top Row"=w303, "Value"=w303, "Item Symbols"=w304) -> ()  [unwired: 2 in, 2 out]
          }
        }
      }
      event "Listbox": Key Down {
        n199 = event-data() -> ("VKey"=w309:T16)  [unwired: 1 in]
        n200 = case shown="\"Left\", \"Right\"" w309 {
          selector: w309 -> [w314 _]
          tunnel: eventvkey."Left" ("VKey") -> [w312 _]
          frame "Left", "Right" {
            n201 = Equal?(x=w312, y=w314) -> (x = y?=w313:bool)
            n202 = Select(t=0, s=w313, f=1) -> (s? t:f=w315:i32)
            n203 = property on="Listbox" class="LstBox (strict)"() -> ("Item Symbols"=w318:i32[])  [unwired: 2 in, 2 out]
            n204 = Replace Array Subset(array=w318, new element=w315, index="Listbox") -> (w317:i32[])
            n205 = property on="Listbox" class="LstBox (strict)"("Item Symbols"=w317) -> ()  [unwired: 2 in, 2 out]
          }
          frame Default {
          }
        }
      }
      event "DB Camera Config": Value Change {
        n206 = event-data() -> ("NewVal"=w322:bool)  [unwired: 1 in]
        n207 = case shown="False" w322 {
          tunnel: w321 -> [w331 _]
          tunnel: [w324 w342] -> w320
          tunnel: w319 -> [w323 w342]
          frame False {
            w338 = "Camera"
            w341 = FALSE ("Visible")
            n208 = local read "Camera Settings"() -> (w330:T2)
            n209 = Index Array(array=w331) -> (element=w334:cluster{string[]})  [unwired: 1 in]
            n210 = Unbundle(w330) -> ("Frame Rate"=w329:i32, "Compression"=w328:i32, "Size"=w332:u16)
            n211 = Unbundle(w334) -> (w333:string[])
            n212 = Index Array(array=w333, index=w332) -> (element=w327:string)
            n213 = call-poly <vilib>:"Write Key.vi"("section"=w338, "value"=w327, "key"="Size", "refnum"=w323) -> ("refnum out"=w340:T15)  [unwired: 2 in, 5 out]
            n214 = call-poly <vilib>:"Write Key.vi"("section"=w338, "value"=w329, "key"="FrameRate", "refnum"=w340) -> ("refnum out"=w339:T15)  [unwired: 1 in, 6 out]
            n215 = property on="Camera Settings" class="Clust (strict)"("Visible"=w341) -> ()  [unwired: 2 in, 2 out]
            n216 = local write "DB Camera Config"(w341) -> ()
            n217 = call-poly <vilib>:"Write Key.vi"("section"=w338, "value"=w328, "key"="Compression", "refnum"=w339) -> ("refnum out"=w325:T15)  [unwired: 1 in, 6 out]
            n218 = call <vilib>:"Close Config Data.vi"("refnum"=w325) -> ("file path"=w326:path)  [unwired: 2 in, 8 out]
            n219 = call <vilib>:"Open Config Data.vi"("configuration file path"=w326) -> ("refnum"=w324:T15)  [unwired: 8 in, 2 out]
          }
          frame True {
            n220 = property on="Camera Settings" class="Clust (strict)"("Visible"=TRUE) -> ()  [unwired: 2 in, 2 out]
          }
        }
      }
      event "Camera Settings": Value Change {
        n221 = event-data() -> ("NewVal"=w355:T2)  [unwired: 1 in]
        n222 = Index Array(array=w351) -> (element=w350:cluster{string[]})  [unwired: 1 in]
        n223 = Unbundle(w355) -> ("Frame Rate"=w346:i32, "Compression"=w345:i32, "Size"=w348:u16)
        n224 = Unbundle(w350) -> (w349:string[])
        n225 = Index Array(array=w349, index=w348) -> (element=w347:string)
        n226 = Format Into String(format string="%s   %dfps   %d%%", w347, w346, w345) -> (resulting string=w352:string)  [unwired: 2 in, 1 out]
        n227 = Build Array(w352) -> (w353:string[])
        n228 = property on="DB Camera Config" class="Bool (strict)"("Strings [4]"=w353) -> ()  [unwired: 2 in, 2 out]
      }
      event "Motor.Enable": Value Change {
        n229 = event-data() -> ("NewVal"=w361:bool)  [unwired: 1 in]
        n230 = Unbundle("Motor") -> ("Value"=w360:dbl)  [unwired: 1 out]
        n231 = Select(t=w360, s=w361, f=0.0) -> (s? t:f=w358:dbl)
        n232 = call <vilib>:"NT Write Number.vi"("Numeric"=w358, "Name"=w357) -> ()  [unwired: 9 in, 1 out]
      }
      event "Test Slider": Value Change {
        n233 = event-data() -> ("NewVal"=w364:dbl)  [unwired: 1 in]
        n234 = call <vilib>:"NT Write Number.vi"("Numeric"=w364, "Name"=w365) -> ()  [unwired: 9 in, 1 out]
      }
      event "On/Off": Value Change {
        n235 = event-data() -> ("NewVal"=w369:bool)  [unwired: 1 in]
        n236 = Boolean To (0,1)(Boolean=w369) -> (0, 1=w368:i16)
        n237 = call <vilib>:"NT Write Number.vi"("Numeric"=w368, "Name"=w367) -> ()  [unwired: 9 in, 1 out]
      }
      event "Rev/Fwd": Value Change {
        n238 = event-data() -> ("NewVal.Forward"=w377:bool, "NewVal.Reverse"=w376:bool)  [unwired: 1 in]
        n239 = Boolean To (0,1)(Boolean=w377) -> (0, 1=w373:i16)
        n240 = Boolean To (0,1)(Boolean=w376) -> (0, 1=w375:i16)
        n241 = Negate(x=w375) -> (-x=w374:i16)
        n242 = Add(x=w373, y=w374) -> (x+y=w372:i16)
        n243 = call <vilib>:"NT Write Number.vi"("Numeric"=w372, "Name"=w371) -> ()  [unwired: 9 in, 1 out]
      }
      event "Test Ring": Value Change {
        n244 = event-data() -> ("NewVal"=w381:u16)  [unwired: 1 in]
        n245 = property on="Test Ring" class="Ring (strict)"() -> ("Strings []"=w382:string[])  [unwired: 2 in, 2 out]
        n246 = Index Array(array=w382, index=w381) -> (element=w380:string)
        n247 = call <vilib>:"NT Write String.vi"("String"=w380, "Name"=w379) -> ()  [unwired: 9 in, 1 out]
      }
      event "Rec Mode": Value Change {
        # "Update globals for recording mode and path to read log from.\nClear when logging and let NetworkTables set path for vision to\nuse."
        n248 = event-data() -> ("NewVal"=w392:enum32{"Stop", "Record", "Playback"})  [unwired: 1 in]
        n249 = global write "WPI_DashboardLogging Global.vi" "Logging Filename"(path "") -> ()
        n250 = case shown="\"Stop\", \"Record\"" w392 {
          tunnel: w391 -> [_ w394 w402]
          tunnel: [_ _ w401] -> w388
          tunnel: [_ _ w400] -> _
          tunnel: w386 -> [_ _ w398]
          tunnel: cluster{i32, i32} {-250, 170} -> [_ _ w397]
          tunnel: [_ _ T17 {"Image Size"=TRUE, "Image Type"=TRUE, "Pixel Value"=TRUE, "ROI Information"=TRUE, "Zoom Factor"=FALSE} ("Image Information Shown:All Elements")] -> w384
          tunnel: [_ _ TRUE ("Zoom Factor")] -> w383
          frame Default {
          }
          frame "Stop", "Record" {
            # "Place Window too"
            n251 = invoke class="VI" method="FP.Close"(reference=w394) -> (reference out=w393:refnum<vi>)  [unwired: 2 in, 2 out]
            n252 = invoke class="VI" method="Abort VI"(reference=w393) -> ()  [unwired: 2 in, 3 out]
          }
          frame "Playback" {
            n253 = call "Open Playback Panel.vi"("Offset"=w397, "DB VI Ref"=w398, "Playback in"=w402) -> ("Playback out"=w399:refnum<vi>)  [unwired: 8 in]
            n254 = register-events(w399) -> (reference out=w401:refnum<event-registration>, error out=w400:errorcluster)  [unwired: 2 in]
          }
        }
        n255 = global write "WPI_DashboardLogging Global.vi" "Recording"(w392) -> ()
        n256 = property on="Camera Image" class="ImageControl"("Image Information Shown"=w384, "Image Information Visible"=w383) -> ()  [unwired: 2 in, 2 out]
        n257 = call <vilib>:"WPI_DashboardNT Log FieldName Cache.vi"("Operation"=enum16{"Lookup/Add", "Index", "Clear"}."Clear") -> ()  [unwired: 8 in, 3 out]
      }
      event Panel Close {
        w403 = enum32{"Stop", "Record", "Playback"}."Stop" ("Rec Mode")
        n258 = event-data() -> ()  [unwired: 1 in, 4 out]
        n259 = local write "Rec Mode"(w403) -> ()
        n260 = global write "WPI_DashboardLogging Global.vi" "Recording"(w403) -> ()
      }
      event Panel Close {
        # "Abort playback window and ourself"
        n261 = event-data() -> ()  [unwired: 1 in, 4 out]
        n262 = invoke class="VI" method="FP.Close"(reference=w408) -> (reference out=w407:refnum<vi>)  [unwired: 2 in, 2 out]
        n263 = invoke class="VI" method="Abort VI"(reference=w407) -> (error out=w406:errorcluster)  [unwired: 2 in, 2 out]
        n264 = invoke class="VI" method="Abort VI"(error in=w406) -> ()  [unwired: 2 in, 3 out]
      }
    }
  }
  n265 = property on="On/Off" class="Bool (strict)"("Visible"=w24) -> ()  [unwired: 2 in, 2 out]
  n266 = property on="Motor" class="Clust (strict)"("Visible"=w24) -> ()  [unwired: 2 in, 2 out]
  n267 = property on="Progress" class="Clust (strict)"("Visible"=w24) -> ()  [unwired: 2 in, 2 out]
  n268 = property on="Test Ring" class="Ring (strict)"("Visible"=w24) -> ()  [unwired: 2 in, 2 out]
  n269 = property on="Rev/Fwd" class="Clust (strict)"("Visible"=w24) -> ()  [unwired: 2 in, 2 out]
  n270 = property on="Camera Settings" class="Clust (strict)"("Visible"=w24) -> ()  [unwired: 2 in, 2 out]
  n271 = local write "DB Camera Config"(w24) -> ()
  n272 = global write "WPI_DashboardLogging Global.vi" "Recording"(w7) -> ()
  n273 = local write "Rec Mode"(w7) -> ()
